vi "Get Or Create Typedef.vi"(8 "error in (no error)":errorcluster, 9 "Create cluster inside Typedef?":bool, 10 "Name":string, 11 "Library in":refnum<vi>) -> (0 "error out":errorcluster, 1 "Cluster ref out":refnum<vi>, 2 "VI ref out":refnum<vi>, 3 "Library out":refnum<vi>, 5 "Path":path)   [LabVIEW 2019, in "gRPC Template Creation Utility.lvlib"]
uses:
  gRPC Template Creation Utility.lvlib
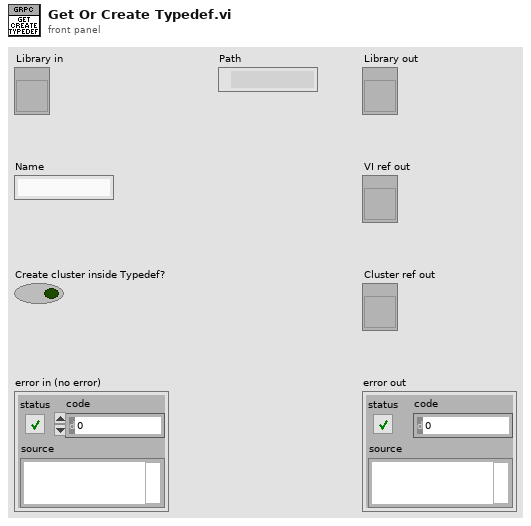
[diagram p1: front panel]
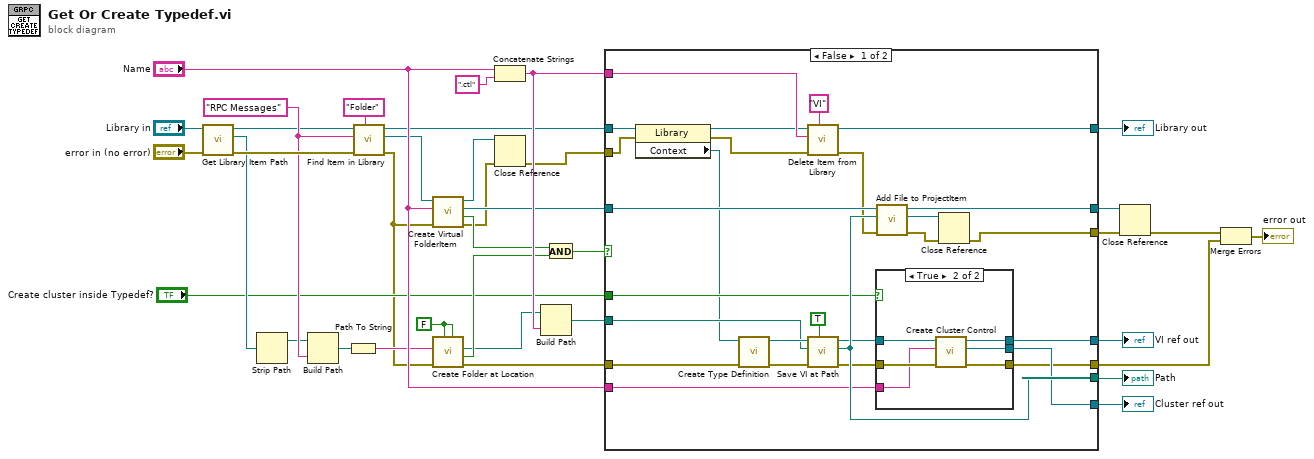
[diagram p0: block diagram]
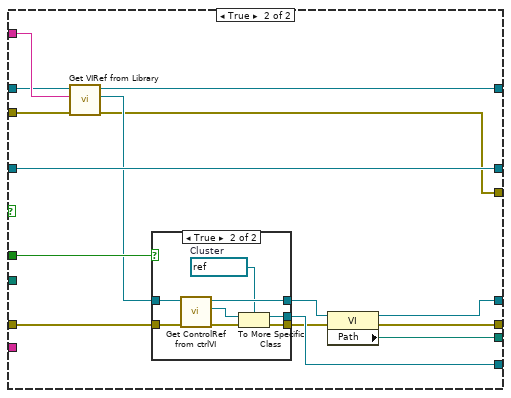
[diagram p3: hidden frame]
diagram:
  w22 = "RPC Messages" ("Item Name")
  w6 = FALSE ("Use Relative")
  n1 = call "Get Library Item Path.vi"("error in (no error)"="error in (no error)", "Library"="Library in") -> ("error out"=w23:errorcluster, "Path"=w16:path, "Library"=w21:refnum<vi>)  [unwired: 7 in]
  n2 = Strip Path(path=w16) -> (stripped path=w15:path)  [unwired: 1 out]
  n3 = Build Path(base path=w15, name or relative path=w22) -> (appended path=w36:path)
  n4 = Path To String(path=w36) -> (string=w13:string)
  n5 = call "Find Item in Library.vi"("Item Type"="Folder", "error in (no error)"=w23, "Item Name"=w22, "Library item in"=w21) -> ("error out"=w1:errorcluster, "Project Item (Library Item)"=w20:refnum<vi>, "Library item out"=w27:refnum<vi>)  [unwired: 4 in, 1 out]
  n6 = call "Create Virtual FolderItem.vi"("error in (no error)"=w1, "Folder Name"="Name", "ProjectItem in"=w20) -> ("error out"=w4:errorcluster, "Already exists?"=w30:bool, "FolderItem reference out"=w26:refnum<vi>, "ProjectItem out"=w3:refnum<vi>)  [unwired: 5 in]
  n7 = call "Create Folder at Location.vi"("Override existing (F)"=w6, "Use Relative (F)"=w6, "Error In"=w1, "Path"=w13) -> ("Error Out"=w14:errorcluster, "Already Exists ?"=w31:bool, "Full path out"=w12:path)  [unwired: 5 in]
  n8 = Concatenate Strings("Name", ".ctl" ("string")) -> (w34:string)
  n9 = Close Reference(reference=w3, error in (no error)=w4) -> (error out=w2:errorcluster)
  n10 = Build Path(base path=w12, name or relative path=w34) -> (appended path=w25:path)
  n11 = And(x=w30, y=w31) -> (x .and. y?=w32:bool)
  n12 = case shown="False" w32 {
    tunnel: w14 -> [w64 w75]
    tunnel: [w46 w85] -> w18
    tunnel: [w63 w78] -> w37
    tunnel: [w62 w73] -> w9
    tunnel: w25 -> [w60 _]
    tunnel: w26 -> [w58 w83]
    tunnel: w27 -> [w42 w82]
    tunnel: [w43 w87] -> w28
    tunnel: [w56 w83] -> w11
    tunnel: w34 -> [w51 w84]
    tunnel: [w57 w86] -> w29
    tunnel: w2 -> [w40 w76]
    tunnel: [w55 w74] -> w10
    tunnel: "Name" -> [w48 _]
    tunnel: "Create cluster inside Typedef?" -> [w47 w81]
    frame False {
      n13 = property class="Library"(reference=w42, error in=w40) -> (reference out=w41:refnum<vi>, error out=w39:errorcluster, "Context"=w38:refnum<vi>)
      n14 = call "Create Type Definition.vi"("error in (no error)"=w64, "application"=w38) -> ("error out"=w59:errorcluster, "TypeDef VI out"=w61:refnum<vi>)  [unwired: 8 in]
      n15 = call "Delete Item from Library.vi"("Item Type"="VI", "error in (no error)"=w39, "Item name"=w51, "Library"=w41) -> ("error out"=w50:errorcluster, "Library"=w43:refnum<vi>)  [unwired: 5 in, 1 out]
      n16 = call "Save VI at Path.vi"("Override Existing? (T)"=TRUE, "error in (no error)"=w59, "Path"=w60, "VI in"=w61) -> ("error out"=w54:errorcluster, "Path to saved File"=w57:path, "VI out"=w53:refnum<vi>)  [unwired: 5 in]
      n17 = case shown="True" w47 {
        tunnel: [_ w72] -> w63
        tunnel: [w66 w71] -> w62
        tunnel: w54 -> [w66 w70]
        tunnel: w53 -> [w65 w69]
        tunnel: w48 -> [_ w68]
        tunnel: [w65 w67] -> w46
        frame False {
        }
        frame True {
          n18 = call "Create Cluster Control.vi"("error in (no error)"=w70, "Cluster Label"=w68, "Owning vi in"=w69) -> ("error out"=w71:errorcluster, "Cluster ref out"=w72:refnum<vi>, "Owning vi out"=w67:refnum<vi>)  [unwired: 6 in]
        }
      }
      n19 = call "Add File to ProjectItem.vi"("error in (no error)"=w50, "File Path"=w57, "ProjectItem in"=w58) -> ("error out"=w44:errorcluster, "Added File ref"=w45:refnum<vi>, "ProjectItem out"=w56:refnum<vi>)  [unwired: 6 in]
      n20 = Close Reference(reference=w45, error in (no error)=w44) -> (error out=w55:errorcluster)
    }
    frame True {
      n21 = call "Get VIRef from Library.vi"("error in (no error)"=w76, "Item Name"=w84, "Library"=w82) -> ("error out"=w74:errorcluster, "VIref out"=w80:refnum<vi>, "Library"=w87:refnum<vi>)  [unwired: 5 in, 1 out]
      n22 = case shown="True" w81 {
        tunnel: w75 -> [w88 w97]
        tunnel: w80 -> [w89 w96]
        tunnel: [w89 w94] -> w79
        tunnel: [_ w91] -> w78
        tunnel: [w88 w90] -> w77
        frame False {
        }
        frame True {
          w93 = refnum<vi> refnum  # Cluster
          n23 = call "Get ControlRef from ctrlVI.vi"("error in (no error)"=w97, "VI ref in"=w96) -> ("error out"=w95:errorcluster, "Control ref out"=w92:refnum<vi>, "VI ref out"=w94:refnum<vi>)  [unwired: 7 in]
          n24 = To More Specific Class(target class=w93, reference=w92, error in=w95) -> (specific class reference=w91:refnum<vi>, error out=w90:errorcluster)
        }
      }
      n25 = property class="VI"(reference=w79, error in=w77) -> (reference out=w85:refnum<vi>, error out=w73:errorcluster, "Path"=w86:path)
    }
  }
  "Cluster ref out" <- w37
  "Path" <- w29
  "Library out" <- w28
  "VI ref out" <- w18
  n26 = Close Reference(reference=w11, error in (no error)=w10) -> (error out=w5:errorcluster)
  n27 = Merge Errors(w5, w9) -> (→"error out":errorcluster)
